vi "Configure daqmx.vi"(8 "error in (no error)":errorcluster, 11 "measurement configuration":T1 {"TYPE" items=["CAN Data"=0, "CAN Remote"=1, "CAN Bus Error"=2, "CAN 2.0 Data"=8, "CAN FD Data"=16, "CAN FD+BRS Data"=24, "J1939 Data"=192, "Delay"=224, "Log Trigger"=225, "Start Trigger"=226]; "PAYLOAD" format="%x"; "IDENTIFIER" format="%x"; "Baudrate" format="%x"; "FD Baudrate" format="%x"; "Active Edge" items=["Rising"=10280, "Falling"=10171]}) -> (0 "error out":errorcluster, 2 "Task out DI":refnum<k21>, 3 "Task out":refnum<k21>)   [LabVIEW 2025]
uses:
  Measurement Configuration.ctl
  <vilib>/DAQmx/create/channels.llb/DAQmx Create Channel (CI-Count Edges).vi
  <resource>/objmgr/daqmx.rc
  <vilib>/DAQmx/create/channels.llb/DAQmx Create Channel (DI-Digital Input).vi
  Workflow DO.lvclass
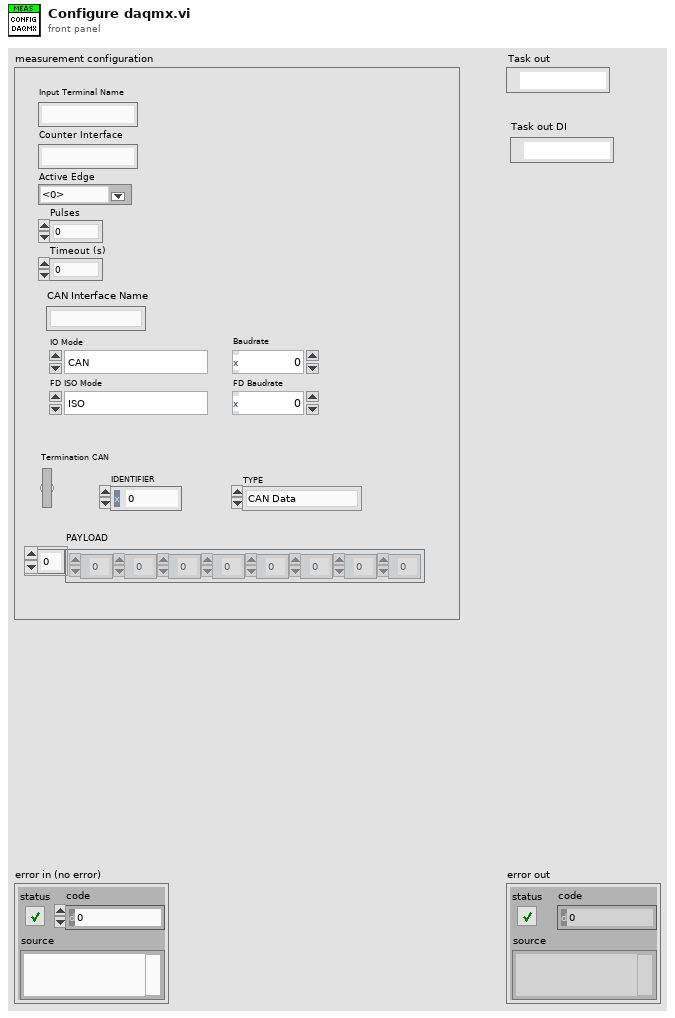
[diagram p1: front panel]
types:
  T1 = typedef "Workflow DO.lvclass/Measurement Configuration.ctl" = cluster{"Input Terminal Name":string, "Counter Interface":string, "Active Edge":i32, "Pulses":u32, "Timeout (s)":u32, "FD Baudrate":u32, "Baudrate":u32, "FD ISO Mode":enum32{"ISO", "Legacy ISO", "Non-ISO"}, "IO Mode":enum32{"CAN", "CAN FD", "CAN FD + BRS"}, "CAN Interface Name":string, "Termination CAN":bool, "IDENTIFIER":u32, "PAYLOAD":u32[], "TYPE":u32}
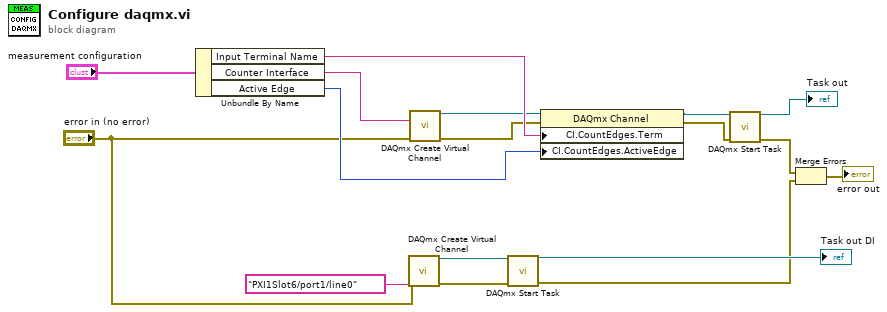
[diagram p0: block diagram]
diagram:
  n1 = Unbundle By Name("measurement configuration") -> ("Input Terminal Name"=w12:string, "Counter Interface"=w13:string, "Active Edge"=w14:i32)
  n2 = call-poly <vilib>:"DAQmx Create Virtual Channel.vi"("lines"=tag "PXI1Slot6/port1/line0" ("Line(s)"), "error in"="error in (no error)") -> ("task out"=w6:refnum<k21>, "error out"=w7:errorcluster)  [unwired: 12 in]
  n3 = call-poly <vilib>:"DAQmx Create Virtual Channel.vi"("counter"=w13, "error in"="error in (no error)") -> ("task out"=w9:refnum<k21>, "error out"=w10:errorcluster)  [unwired: 12 in]
  n4 = call <vilib>:"DAQmx Start Task.vi"("task/channels in"=w6, "error in"=w7) -> ("task out"=→"Task out DI":refnum<k21>, "error out"=w2:errorcluster)  [unwired: 12 in]
  n5 = property class="DAQmx Channel"(reference=w9, error in=w10, "CI.CountEdges.Term"=w12, "CI.CountEdges.ActiveEdge"=w14) -> (reference out=w15:refnum<k21>, error out=w17:errorcluster)
  n6 = call <vilib>:"DAQmx Start Task.vi"("task/channels in"=w15, "error in"=w17) -> ("task out"=→"Task out":refnum<k21>, "error out"=w3:errorcluster)  [unwired: 12 in]
  n7 = Merge Errors(w3, w2) -> (→"error out":errorcluster)
